vi "AlliGator Get All Graph Refnums.vi"(8 "Error In":errorcluster) -> (0 "Error Out":errorcluster, 3 "All Graph Refnums":refnum<vi>[](array[refnum]))   [LabVIEW 2021, in "AlliGator GUI.lvlib"]
uses:
  AlliGator GUI.lvlib
  Image Histogram/AlliGator Image Histogram Control Refnums.ctl
  Globals, Variables, Constants/AlliGator Refnums List.ctl
  Intensity Time Trace/AlliGator Intensity Time Trace Ctrl Refnums.ctl
  Decay Graph/AlliGator Decay Graph Ctrl Refnums.ctl
  Decay Statistics/AlliGator Decay Statistics Graph Ctrl Refnums.ctl
  Phasor Graph/AlliGator Phasor Graph Ctrl Refnums.ctl
  Phasor Ratio/AlliGator Phasor Ratio Graph Ctrl Refnums.ctl
  Lifetime & Other Parameters/AlliGator Lifetime & Other Parameters Ctrl Refnums.ctl
  Image Histogram/AlliGator Image Histogram.lvlib
  Intensity Time Trace/AlliGator Intensity Time Trace.lvlib
  Decay Graph/AlliGator Decay Graph.lvlib
  Decay Statistics/AlliGator Decay Statistics.lvlib
  Phasor Graph/AlliGator Phasor Graph.lvlib
  Phasor Ratio/AlliGator Phasor Ratio.lvlib
  Lifetime & Other Parameters/AlliGator Lifetime & Other Parameters.lvlib
panel:
  # "see the License on the block diagram (Ctrl+E or Window:Show Block Diagram)"
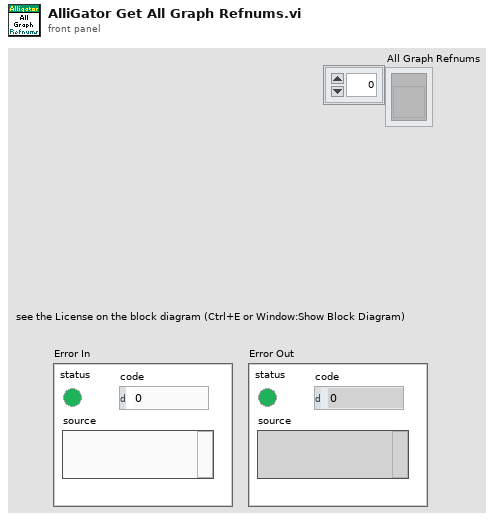
[diagram p1: front panel]
types:
  T1 = typedef "AlliGator Lifetime & Other Parameters.lvlib/AlliGator Lifetime & Other Parameters Ctrl Refnums.ctl" = cluster{"Lifetime Graph":refnum<vi>}
  T2 = typedef "AlliGator Phasor Ratio.lvlib/AlliGator Phasor Ratio Graph Ctrl Refnums.ctl" = cluster{"Phasor Ratio Graph":refnum<vi>}
  T3 = typedef "AlliGator Phasor Graph.lvlib/AlliGator Phasor Graph Ctrl Refnums.ctl" = cluster{"Phasor Ratio":refnum<vi>, "Modulus Lifetime":refnum<vi>, "Phasor at cursor (m, phi)":refnum<vi>, "Phase Lifetime":refnum<vi>, "Phasor at cursor (g, s)":refnum<vi>, "Phasor Graph Average Lifetime":refnum<vi>, "Phasor Graph Active":refnum<vi>, "Save Phasor Graph":refnum<vi>, "Phasor Frame Slide":refnum<vi>, "Single Step Phasor":refnum<vi>, "Calibration Type":refnum<vi>, "Show Line":refnum<vi>, "Phase Lifetime 1":refnum<vi>, "Phase Lifetime 2":refnum<vi>, "Phasor Graph Frequency":refnum<vi>, "Phasor Reference 1 Control":refnum<vi>, "Phasor Reference 2 Control":refnum<vi>, "Calibration Lifetime":refnum<vi>, "Phase Lifetime SDV":refnum<vi>, "Average Lifetime SDV":refnum<vi>, "Phasor Ratio SDV":refnum<vi>, "Modulus Lifetime SDV":refnum<vi>, "Phasor Graph":refnum<vi>}
  T4 = typedef "AlliGator Decay Statistics.lvlib/AlliGator Decay Statistics Graph Ctrl Refnums.ctl" = cluster{"Decay Statistics Graph":refnum<vi>, "Decay Statistics Bin":refnum<vi>}
  T5 = typedef "AlliGator Decay Graph.lvlib/AlliGator Decay Graph Ctrl Refnums.ctl" = cluster{"Decay Graph":refnum<vi>, "Decay Graph Active":refnum<vi>}
  T6 = typedef "AlliGator Intensity Time Trace.lvlib/AlliGator Intensity Time Trace Ctrl Refnums.ctl" = cluster{"Intensity Time Trace":refnum<vi>, "Time Step":refnum<vi>, "Use File Timestamp":refnum<vi>}
  T7 = typedef "AlliGator GUI.lvlib/AlliGator Refnums List.ctl" = enum16{"---------- AlliGator Control Refnums ----------", "AlliGator Tab Control Refnum", "Dataset Ctrl Refnums", "Image Histogram Ctrl Refnums", "Intensity Time Trace Ctrl Refnums", "Decay Graph Ctrl Refnums", "Decay Statistics Graph Ctrl Refnums", "Phasor Graph Ctrl Refnums", "Phasor Ratio Graph Ctrl Refnums", "Phasor Plot Ctrl Refnums", "Lifetime & Other Parameters Ctrl Refnums", "Decay Fit Parameter Map Ctrl Refnums", "Parameter Map Ctrl Refnums", "Other AlliGator Ctrl Refnums", "---------- AlliGator Menu Refnums ----------", "AlliGator Menu", "---------- AlliGator VI Refnums ----------", "AlliGator Refnum", "AlliGator Settings Refnum", "AlliGator Launcher Refnum", "---------- IO Device ID ----------", "Mouse ID", "Keyboard ID"}
  T8 = typedef "AlliGator Image Histogram.lvlib/AlliGator Image Histogram Control Refnums.ctl" = cluster{"Image Histogram":refnum<vi>, "Image Histogram Options":refnum<vi>, "Image Histogram Active":refnum<vi>, "Image Histogram Upper Percentile":refnum<vi>, "Image Histogram Lower Percentile":refnum<vi>, "Auto-Adjust Contrast":refnum<vi>}
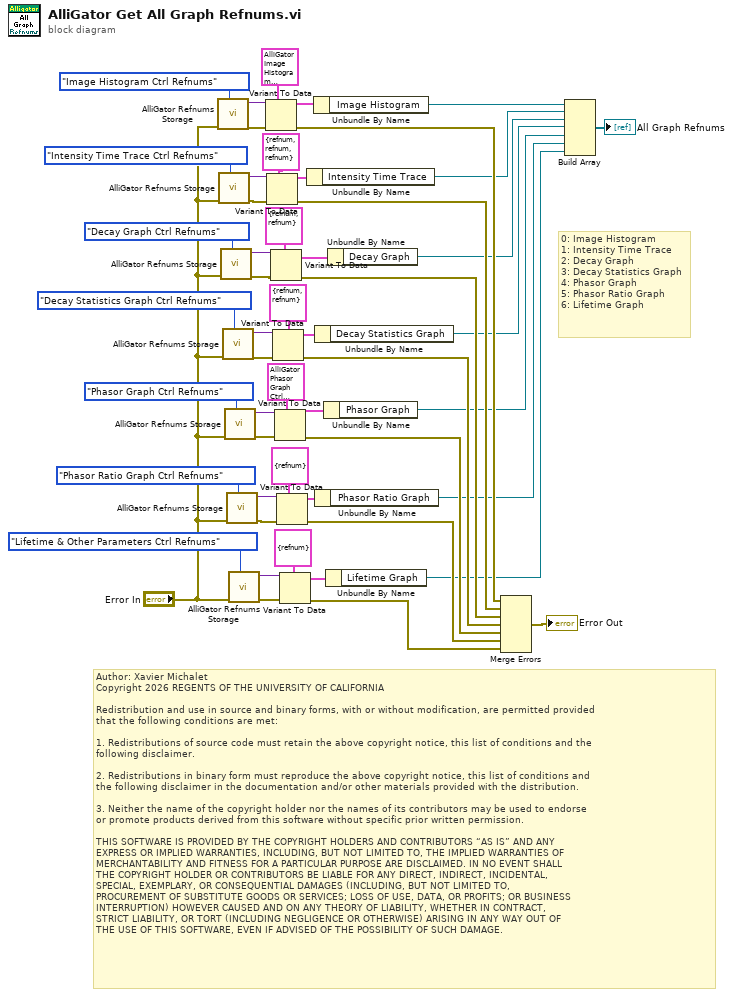
[diagram p0: block diagram]
diagram:
  # "0: Image Histogram\n1: Intensity Time Trace\n2: Decay Graph\n3: Decay Statistics Graph\n4: Phasor Graph\n5: Phasor Ratio Graph\n6: Lifetime Graph"
  # "Author: Xavier Michalet\nCopyright 2026 REGENTS OF THE UNIVERSITY OF CALIFORNIA\n\nRedistribution and use in source and binary forms, with or without modification, are permitted provided\nthat the following conditions are met:\n\n1. Redistributions of source code must retain the above copyright notice, this list of conditions and the\nfollowing disclaimer.\n\n2. Redistributions in binary form must reproduce the above copyright notice, this list of conditions and\nthe following disclaimer in the documentation and/or other materials provided with the distribution.\n\n3. Neither the name of the copyright holder nor the names of its contributors may be used to endorse \nor promote products derived from this software without specific prior written permission.\n\nTHIS SOFTWARE IS PROVIDED BY THE COPYRIGHT HOLDERS AND CONTRIBUTORS “AS IS” AND ANY \nEXPRESS OR IMPLIED WARRANTIES, INCLUDING, BUT NOT LIMITED TO, THE IMPLIED WARRANTIES OF\nMERCHANTABILITY AND FITNESS FOR A PARTICULAR PURPOSE ARE DISCLAIMED. IN NO EVENT SHALL\nTHE COPYRIGHT HOLDER OR CONTRIBUTORS BE LIABLE FOR ANY DIRECT, INDIRECT, INCIDENTAL, \nSPECIAL, EXEMPLARY, OR CONSEQUENTIAL DAMAGES (INCLUDING, BUT NOT LIMITED TO, \nPROCUREMENT OF SUBSTITUTE GOODS OR SERVICES; LOSS OF USE, DATA, OR PROFITS; OR BUSINESS\nINTERRUPTION) HOWEVER CAUSED AND ON ANY THEORY OF LIABILITY, WHETHER IN CONTRACT, \nSTRICT LIABILITY, OR TORT (INCLUDING NEGLIGENCE OR OTHERWISE) ARISING IN ANY WAY OUT OF\nTHE USE OF THIS SOFTWARE, EVEN IF ADVISED OF THE POSSIBILITY OF SUCH DAMAGE."
  n1 = call "AlliGator Refnums Storage.vi"("AlliGator Refnum List"=AlliGator_Refnums_List."Image Histogram Ctrl Refnums", "Error In"="Error In") -> ("Error Out"=w50:errorcluster, "Data out"=w51:variant)  [unwired: 8 in]
  n2 = call "AlliGator Refnums Storage.vi"("AlliGator Refnum List"=AlliGator_Refnums_List."Intensity Time Trace Ctrl Refnums", "Error In"="Error In") -> ("Error Out"=w18:errorcluster, "Data out"=w49:variant)  [unwired: 8 in]
  n3 = call "AlliGator Refnums Storage.vi"("AlliGator Refnum List"=AlliGator_Refnums_List."Decay Graph Ctrl Refnums", "Error In"="Error In") -> ("Error Out"=w19:errorcluster, "Data out"=w48:variant)  [unwired: 8 in]
  n4 = call "AlliGator Refnums Storage.vi"("AlliGator Refnum List"=AlliGator_Refnums_List."Decay Statistics Graph Ctrl Refnums", "Error In"="Error In") -> ("Error Out"=w20:errorcluster, "Data out"=w46:variant)  [unwired: 8 in]
  n5 = call "AlliGator Refnums Storage.vi"("AlliGator Refnum List"=AlliGator_Refnums_List."Phasor Graph Ctrl Refnums", "Error In"="Error In") -> ("Error Out"=w21:errorcluster, "Data out"=w47:variant)  [unwired: 8 in]
  n6 = call "AlliGator Refnums Storage.vi"("AlliGator Refnum List"=AlliGator_Refnums_List."Phasor Ratio Graph Ctrl Refnums", "Error In"="Error In") -> ("Error Out"=w22:errorcluster, "Data out"=w45:variant)  [unwired: 8 in]
  n7 = call "AlliGator Refnums Storage.vi"("AlliGator Refnum List"=AlliGator_Refnums_List."Lifetime & Other Parameters Ctrl Refnums", "Error In"="Error In") -> ("Error Out"=w23:errorcluster, "Data out"=w44:variant)  [unwired: 8 in]
  n8 = Variant To Data(error in=w50, type=T8 {"Image Histogram"=refnum, "Image Histogram Options"=refnum, "Image Histogram Active"=refnum, "Image Histogram Upper Percentile"=refnum, "Image Histogram Lower Percentile"=refnum, "Auto-Adjust Contrast"=refnum} ("Image Histogram Ctrl Refnums"), Variant=w51) -> (data=w42:T8, error out=w15:errorcluster)
  n9 = Variant To Data(error in=w18, type=T6 {"Intensity Time Trace"=refnum, "Time Step"=refnum, "Use File Timestamp"=refnum} ("Intensity Time Trace Ctrl Refnums"), Variant=w49) -> (data=w39:T6, error out=w14:errorcluster)
  n10 = Variant To Data(error in=w19, type=T5 {"Decay Graph"=refnum, "Decay Graph Active"=refnum} ("Decay Graph Ctrl Refnums"), Variant=w48) -> (data=w33:T5, error out=w13:errorcluster)
  n11 = Variant To Data(error in=w20, type=T4 {"Decay Statistics Graph"=refnum, "Decay Statistics Bin"=refnum} ("Decay Statistics Graph Ctrl Refnums"), Variant=w46) -> (data=w32:T4, error out=w12:errorcluster)
  n12 = Variant To Data(error in=w21, type=T3 {"Phasor Ratio"=refnum, "Modulus Lifetime"=refnum, "Phasor at cursor (m, phi)"=refnum, "Phase Lifetime"=refnum, "Phasor at cursor (g, s)"=refnum, "Phasor Graph Average Lifetime"=refnum, "Phasor Graph Active"=refnum, "Save Phasor Graph"=refnum, "Phasor Frame Slide"=refnum, "Single Step Phasor"=refnum, "Calibration Type"=refnum, "Show Line"=refnum, "Phase Lifetime 1"=refnum, "Phase Lifetime 2"=refnum, "Phasor Graph Frequency"=refnum, "Phasor Reference 1 Control"=refnum, "Phasor Reference 2 Control"=refnum, "Calibration Lifetime"=refnum, "Phase Lifetime SDV"=refnum, "Average Lifetime SDV"=refnum, "Phasor Ratio SDV"=refnum, "Modulus Lifetime SDV"=refnum, "Phasor Graph"=refnum} ("Phasor Graph Ctrl Refnums"), Variant=w47) -> (data=w31:T3, error out=w11:errorcluster)
  n13 = Variant To Data(error in=w22, type=T2 {"Phasor Ratio Graph"=refnum} ("Phasor Ratio Graph Ctrl Refnums"), Variant=w45) -> (data=w30:T2, error out=w10:errorcluster)
  n14 = Variant To Data(error in=w23, type=T1 {"Lifetime Graph"=refnum} ("Lifetime & Other Parameters Graph Ctrl Refnums"), Variant=w44) -> (data=w29:T1, error out=w9:errorcluster)
  n15 = Unbundle By Name(w39) -> ("Intensity Time Trace"=w7:refnum<vi>)
  n16 = Unbundle By Name(w42) -> ("Image Histogram"=w8:refnum<vi>)
  n17 = Unbundle By Name(w32) -> ("Decay Statistics Graph"=w5:refnum<vi>)
  n18 = Unbundle By Name(w30) -> ("Phasor Ratio Graph"=w3:refnum<vi>)
  n19 = Unbundle By Name(w31) -> ("Phasor Graph"=w4:refnum<vi>)
  n20 = Unbundle By Name(w29) -> ("Lifetime Graph"=w2:refnum<vi>)
  n21 = Unbundle By Name(w33) -> ("Decay Graph"=w6:refnum<vi>)
  n22 = Merge Errors(w15, w14, w13, w12, w11, w10, w9) -> (→"Error Out":errorcluster)
  n23 = Build Array(w8, w7, w6, w5, w4, w3, w2) -> (→"All Graph Refnums":refnum<vi>[])
